vi "Remove Panel at Index.vi"(7 "Close Removed (T)":bool=TRUE, 8 "error in (no error)":errorcluster, 9 "2D Index":T1, 11 "2DArrayManager in":refnum<class "2DArrayManager.lvclass">) -> (0 "error out":errorcluster, 1 "Element Removed":bool, 2 "Removed Element":refnum<class "ArrayPanel.lvclass">, 3 "2DArrayManager out":refnum<class "2DArrayManager.lvclass">)   [LabVIEW 2020, in "OOPanel.lvlib" / "2DArrayManager.lvclass"]
uses:
  2DArrayManager.lvclass
  2D Index.ctl
  ArrayPanel/ArrayPanel.lvclass
  C:/dev/lv20CE/relink/lv-oopanel/OOPanel/Panel/Panel.lvclass
  2DArrayManager.lvclass/2DArrayManager.ctl
  ArrayPanel/ArrayPanel.lvclass/ArrayPanel.ctl
  Panel/Panel.lvclass
  Manager/Manager.lvclass
  OOPanel.lvlib
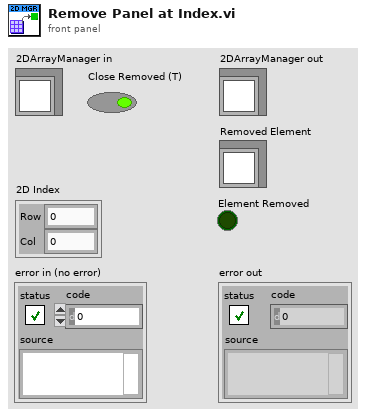
[diagram p1: front panel]
types:
  T1 = typedef "OOPanel.lvlib/2D Index.ctl" = cluster{"Row":i32, "Col":i32}
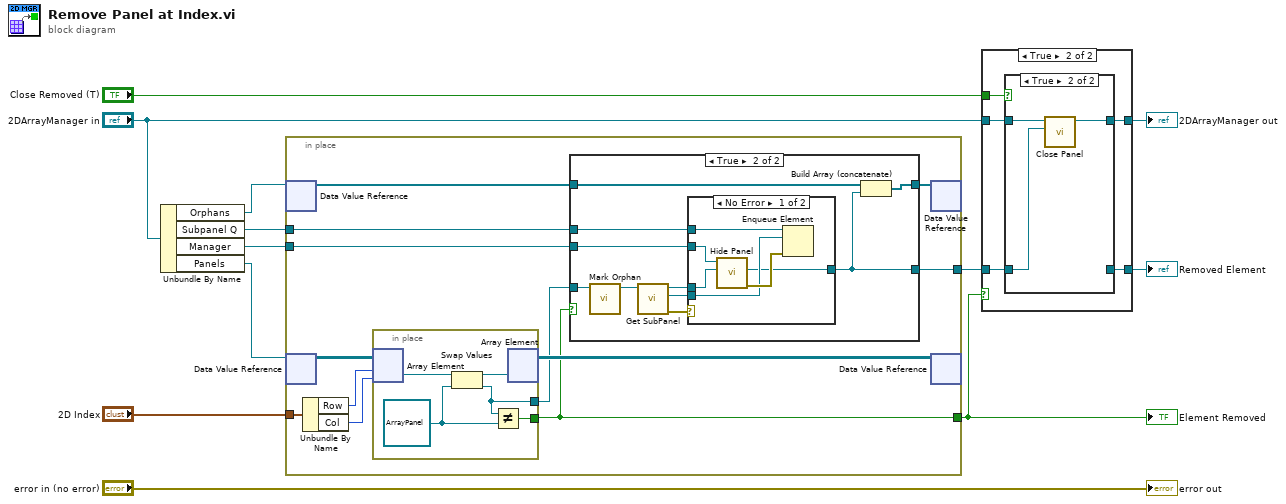
[diagram p0: block diagram]
diagram:
  n1 = Unbundle By Name("2DArrayManager in") -> ("Orphans"=w11:refnum<data-value>, "Subpanel Q"=w2:refnum<queue>, "Manager"=w1:refnum<class "Manager.lvclass">, "Panels"=w10:refnum<data-value>)
  n2 = in-place {
    in-place-border: "2D Index" -> [w23]
    in-place-border: [w18] -> w3
    in-place-border: [w15] -> w5
    in-place-border: w2 -> [w14]
    in-place-border: w1 -> [w13]
    n3 = in-place-dvr #1(w11) -> (w19:refnum<class "ArrayPanel.lvclass">[])  [unwired: 1 out]
    n4 = in-place-dvr #2(w10) -> (w24:refnum<class "ArrayPanel.lvclass">[][])  [unwired: 1 out]
    n5 = Unbundle By Name(w23) -> ("Row"=w22:i32, "Col"=w21:i32)
    n6 = in-place {
      in-place-border: [w26] -> w18
      in-place-border: [w25] -> w17
      w27 = refnum<class "ArrayPanel.lvclass"> refnum ("element")
      n7 = in-place-array #3(w24, w22, w21) -> (w29:refnum<class "ArrayPanel.lvclass">)
      n8 = Swap Values(12:w29, 14:w27) -> (1:w28:refnum<class "ArrayPanel.lvclass">, 3:w25:refnum<class "ArrayPanel.lvclass">)  [unwired: 1 in]
      n9 = Not Equal?(x=w25, y=w27) -> (x != y?=w26:bool)
      n10 = in-place-array #3(w28) -> (w20:refnum<class "ArrayPanel.lvclass">[][])  [unwired: 2 out]
    }
    n11 = case shown="True" w18 {
      tunnel: w19 -> [w30 w40]
      tunnel: w17 -> [_ w39]
      tunnel: [w30 w38] -> w16
      tunnel: [_ w31] -> w15
      tunnel: w14 -> [_ w32]
      tunnel: w13 -> [_ w33]
      frame False {
      }
      frame True {
        n12 = call "Mark Orphan.vi"("ArrayPanel in"=w39) -> ("ArrayPanel out"=w37:refnum<class "ArrayPanel.lvclass">)  [unwired: 9 in, 1 out]
        n13 = call "Get SubPanel.vi"("Panel in"=w37) -> ("error out"=w36:errorcluster, "SubPanel"=w35:refnum<vi>, "Panel out"=w34:refnum<class "ArrayPanel.lvclass">)  [unwired: 8 in]
        n14 = case shown="No Error" w36 {
          tunnel: w35 -> [w42 _]
          tunnel: w34 -> [w45 w47]
          tunnel: w33 -> [w44 _]
          tunnel: w32 -> [w43 _]
          tunnel: [w41 w47] -> w31
          frame No Error {
            n15 = call "Hide Panel.vi"("Panel In"=w45, "Manager in"=w44) -> ("error out"=w46:errorcluster, "Panel"=w41:refnum<class "ArrayPanel.lvclass">)  [unwired: 7 in, 1 out]
            n16 = Enqueue Element(queue=w43, element=w42, error in (no error)=w46) -> ()  [unwired: 1 in, 3 out]
          }
          frame Error {
          }
        }
        n17 = Build Array (concatenate)(w40, w31) -> (w38:refnum<class "ArrayPanel.lvclass">[])
      }
    }
    n18 = in-place-dvr #1(w16) -> ()  [unwired: 2 out]
    n19 = in-place-dvr #2(w20) -> ()  [unwired: 2 out]
  }
  "Element Removed" <- w3
  n20 = case shown="True" w3 {
    tunnel: w5 -> [_ w53]
    tunnel: [_ w52] -> w4
    tunnel: "Close Removed (T)" -> [_ w51]
    tunnel: "2DArrayManager in" -> [w48 w50]
    tunnel: [w48 w49] -> w8
    frame False {
    }
    frame True {
      n21 = case shown="True" w51 {
        tunnel: w53 -> [w54 w58]
        tunnel: [w54 _] -> w52
        tunnel: w50 -> [w55 w57]
        tunnel: [w55 w56] -> w49
        frame False {
        }
        frame True {
          n22 = call "Close Panel.vi"("ArrayPanel"=w58, "2DArrayManager in"=w57) -> ("2DArrayManager out"=w56:refnum<class "2DArrayManager.lvclass">)  [unwired: 8 in, 1 out]
        }
      }
    }
  }
  "2DArrayManager out" <- w8
  "Removed Element" <- w4
  "error out" <- "error in (no error)"
